vi "ZM-TST-udp.vi"() -> (0 "error out":errorcluster, 3 "Pass":bool)   [LabVIEW 2020, in "ZM-TST-tests.lvlib"]
doc: "T5, test of the UDP transport and the multi protocol: a sent package arrives unchanged, a receive with no data times out, sending with no listener is silent, a multi protocol of two file loggers writes to both, and publish on the receiver returns 5000. Pass = AND of the six checks. Side effects: UDP on 127.0.0.1:61557, two folders under output."
uses:
  ZM-TST-tests.lvlib
  protocol/ZM-CP-UDP-udp_transport/ZM-CP-UDP-receiver/ZM-CP-UDP-receiver.lvclass
  protocol/ZM-CP-UDP-udp_transport/ZM-CP-UDP-sender/ZM-CP-UDP-sender.lvclass
  protocol/ZM-CP-FL-file_logger/ZM-CP-FL-file_logger/ZM-CP-FL-file_logger.lvclass
  protocol/ZM-CP-communication_protocol/ZM-CP-communication_protocol/ZM-CP-communication_protocol.lvclass
  protocol/ZM-CP-MX-multi_protocol/ZM-CP-MX-multi_protocol/ZM-CP-MX-multi_protocol.lvclass
  common/ZM-PC-packages/ZM-PC-TP-test_package/ZM-PC-TP-test_package.lvclass
  common/ZM-PC-packages/ZM-PC-package/ZM-PC-package.lvclass
panel:
  out "rx_publish_5000_ok":bool
  out "mx_ok":bool
  out "no_listener_ok":bool
  out "timeout_ok":bool
  out "roundtrip_ok":bool
  out "rx_init_ok":bool
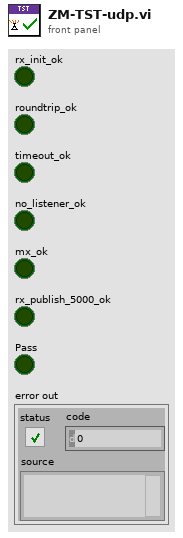
[diagram p1: front panel]
types:
  T1 = cluster{"timestamp":string, "type":string, "destination":string, "data":cluster{"temperature_c":dbl, "sample_index":i32, "duty_percent":u8, "sensor_ok":bool, "status":string}}
  T2 = enum16{"Unknown", "Root", "Hardware", "Communication"}
  T3 = cluster{"temperature_c":dbl, "sample_index":i32, "duty_percent":u8, "sensor_ok":bool, "status":string}
  T4 = cluster{"temperature_c":bool, "sample_index":bool, "duty_percent":bool, "sensor_ok":bool, "status":bool}
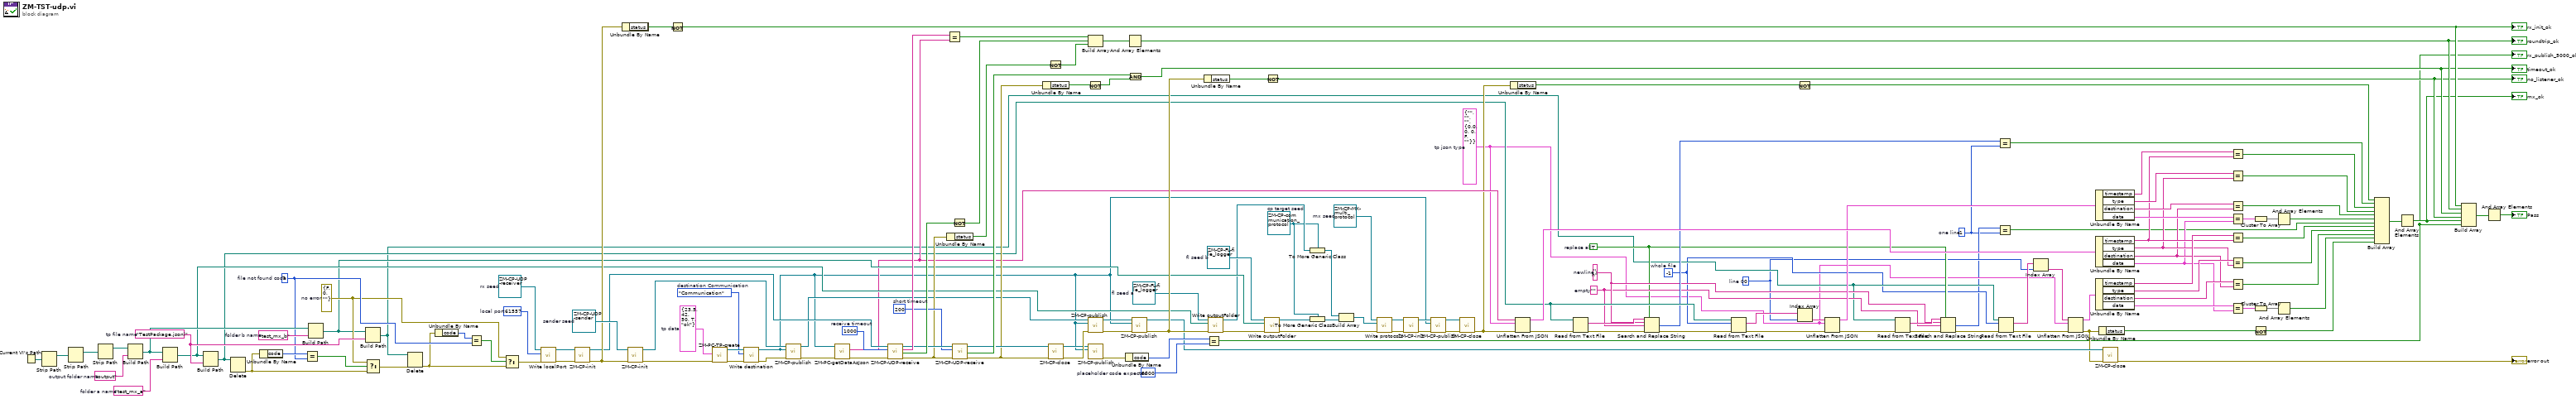
[diagram p0: block diagram]
diagram:
  w12 = 5000  # placeholder code expected
  w47 = 0  # line 0
  w41 = 1  # one line
  w50 = -1  # whole file
  w52 = TRUE  # replace all
  w54 = ""  # empty
  w55 = "\n"  # newline
  w45 = T1 {"timestamp"="", "type"="", "destination"="", "data"={"temperature_c"=0.0, "sample_index"=0, "duty_percent"=0, "sensor_ok"=FALSE, "status"=""}}  # tp json type
  w139 = errorcluster {"status"=FALSE, "code"=0, "source"=""}  # no error
  w140 = 7  # file not found code
  w146 = "TestPackage.jsonl"  # tp file name
  w147 = "test_mx_b"  # folder b name
  w149 = "test_mx_a"  # folder a name
  w150 = "output"  # output folder name
  w109 = 200  # short timeout
  w119 = 1000  # receive timeout
  w124 = T2."Communication"  # destination Communication
  w128 = T3 {"temperature_c"=23.5, "sample_index"=42, "duty_percent"=50, "sensor_ok"=TRUE, "status"="ok"}  # tp data
  w134 = u16 61557  # local port
  w86 = refnum<class "ZM-CP-MX-multi_protocol.lvclass"> refnum  # mx seed
  w89 = refnum<class "ZM-CP-communication_protocol.lvclass"> refnum  # cp target seed
  w93 = refnum<class "ZM-CP-FL-file_logger.lvclass"> refnum  # fl seed b
  w96 = refnum<class "ZM-CP-FL-file_logger.lvclass"> refnum  # fl seed a
  w130 = refnum<class "ZM-CP-UDP-sender.lvclass"> refnum  # sender seed
  w135 = refnum<class "ZM-CP-UDP-receiver.lvclass"> refnum  # rx seed
  n1 = Current VI's Path() -> (path=w154:path)
  n2 = Strip Path(path=w154) -> (stripped path=w153:path)  [unwired: 1 out]
  n3 = Strip Path(path=w153) -> (stripped path=w152:path)  [unwired: 1 out]
  n4 = Strip Path(path=w152) -> (stripped path=w151:path)  [unwired: 1 out]
  n5 = Build Path(base path=w151, name or relative path=w150) -> (appended path=w148:path)
  n6 = Build Path(base path=w148, name or relative path=w149) -> (appended path=w95:path)
  n7 = Build Path(base path=w95, name or relative path=w146) -> (appended path=w70:path)
  n8 = Delete(path (use dialog)=w70) -> (error out=w143:errorcluster)  [unwired: 4 in, 2 out]
  n9 = Unbundle By Name(w143) -> ("code"=w145:i32)
  n10 = Equal?(x=w145, y=w140) -> (x = y?=w144:bool)
  n11 = Build Path(base path=w148, name or relative path=w147) -> (appended path=w92:path)
  n12 = Build Path(base path=w92, name or relative path=w146) -> (appended path=w51:path)
  n13 = Select(t=w139, s=w144, f=w143) -> (s? t:f=w142:errorcluster)
  n14 = Delete(path (use dialog)=w51, error in=w142) -> (error out=w137:errorcluster)  [unwired: 3 in, 2 out]
  n15 = Unbundle By Name(w137) -> ("code"=w141:i32)
  n16 = Equal?(x=w141, y=w140) -> (x = y?=w138:bool)
  n17 = Select(t=w139, s=w138, f=w137) -> (s? t:f=w136:errorcluster)
  n18 = call "Write localPort.vi"("error in (no error)"=w136, "localPort"=w134, "ZM-CP-UDP-receiver in"=w135) -> ("error out"=w132:errorcluster, "ZM-CP-UDP-receiver out"=w133:refnum<class "ZM-CP-UDP-receiver.lvclass">)  [unwired: 7 in]
  n19 = call-dynamic "ZM-CP-init.vi"("error in (no error)"=w132, "ZM-CP-UDP-receiver in"=w133) -> ("error out"=w129:errorcluster, "ZM-CP-UDP-receiver out"=w120:refnum<class "ZM-CP-UDP-receiver.lvclass">)  [unwired: 8 in]
  n20 = Unbundle By Name(w129) -> ("status"=w131:bool)
  n21 = call-dynamic "ZM-CP-init.vi"("error in (no error)"=w129, "ZM-CP-UDP-sender in"=w130) -> ("error out"=w127:errorcluster, "ZM-CP-UDP-sender out"=w123:refnum<class "ZM-CP-UDP-sender.lvclass">)  [unwired: 8 in]
  n22 = Not(x=w131) -> (.not. x?=w8:bool)
  "rx_init_ok" <- w8
  n23 = call "ZM-PC-TP-create.vi"("error in (no error)"=w127, "data"=w128) -> ("error out"=w126:errorcluster, "package"=w125:refnum<class "ZM-PC-TP-test_package.lvclass">)  [unwired: 8 in]
  n24 = call "Write destination.vi"("error in (no error)"=w126, "ZM-PC-DESTINATION"=w124, "ZM-PC-package in"=w125) -> ("error out"=w122:errorcluster, "ZM-PC-package out"=w15:refnum<class "ZM-PC-TP-test_package.lvclass">)  [unwired: 7 in]
  n25 = call-dynamic "ZM-CP-publish.vi"("error in (no error)"=w122, "package"=w15, "ZM-CP-UDP-sender in"=w123) -> ("error out"=w121:errorcluster, "ZM-CP-UDP-sender out"=w102:refnum<class "ZM-CP-UDP-sender.lvclass">)  [unwired: 7 in]
  n26 = call-dynamic "ZM-PC-getDataAsJson.vi"("error in (no error)"=w121, "ZM-PC-TP-test_package in"=w15) -> ("error out"=w118:errorcluster, "json"=w76:string)  [unwired: 7 in, 1 out]
  n27 = call "ZM-CP-UDP-receive.vi"("error in (no error)"=w118, "timeout_ms"=w119, "ZM-CP-UDP-receiver in"=w120) -> ("error out"=w108:errorcluster, "timed_out"=w116:bool, "json"=w117:string, "ZM-CP-UDP-receiver out"=w110:refnum<class "ZM-CP-UDP-receiver.lvclass">)  [unwired: 5 in]
  n28 = Unbundle By Name(w108) -> ("status"=w115:bool)
  n29 = Equal?(x=w117, y=w76) -> (x = y?=w114:bool)
  n30 = Not(x=w116) -> (.not. x?=w113:bool)
  n31 = call "ZM-CP-UDP-receive.vi"("error in (no error)"=w108, "timeout_ms"=w109, "ZM-CP-UDP-receiver in"=w110) -> ("error out"=w103:errorcluster, "timed_out"=w106:bool, "ZM-CP-UDP-receiver out"=w104:refnum<class "ZM-CP-UDP-receiver.lvclass">)  [unwired: 5 in, 1 out]
  n32 = Unbundle By Name(w103) -> ("status"=w107:bool)
  n33 = Not(x=w115) -> (.not. x?=w112:bool)
  n34 = call-dynamic "ZM-CP-close.vi"("error in (no error)"=w103, "ZM-CP-UDP-receiver in"=w104) -> ("error out"=w101:errorcluster, "ZM-CP-UDP-receiver out"=w16:refnum<class "ZM-CP-UDP-receiver.lvclass">)  [unwired: 8 in]
  n35 = Not(x=w107) -> (.not. x?=w105:bool)
  n36 = Build Array(w114, w113, w112) -> (w111:bool[])
  n37 = call-dynamic "ZM-CP-publish.vi"("error in (no error)"=w101, "package"=w15, "ZM-CP-UDP-sender in"=w102) -> ("error out"=w99:errorcluster, "ZM-CP-UDP-sender out"=w100:refnum<class "ZM-CP-UDP-sender.lvclass">)  [unwired: 7 in]
  n38 = call-dynamic "ZM-CP-publish.vi"("package"=w15, "ZM-CP-communication_protocol in"=w16) -> ("error out"=w14:errorcluster)  [unwired: 8 in, 1 out]
  n39 = Unbundle By Name(w14) -> ("code"=w13:i32)
  n40 = And Array Elements(Boolean array=w111) -> (logical AND=w7:bool)
  "roundtrip_ok" <- w7
  n41 = And(x=w106, y=w105) -> (x .and. y?=w6:bool)
  "timeout_ok" <- w6
  n42 = call-dynamic "ZM-CP-publish.vi"("error in (no error)"=w99, "package"=w15, "ZM-CP-UDP-sender in"=w100) -> ("error out"=w97:errorcluster, "ZM-CP-UDP-sender out"=w11:refnum<class "ZM-CP-UDP-sender.lvclass">)  [unwired: 7 in]
  n43 = Unbundle By Name(w97) -> ("status"=w98:bool)
  n44 = Equal?(x=w13, y=w12) -> (x = y?=w3:bool)
  "rx_publish_5000_ok" <- w3
  n45 = call "Write outputFolder.vi"("error in (no error)"=w97, "outputFolder"=w95, "ZM-CP-FL-file_logger in"=w96) -> ("error out"=w94:errorcluster, "ZM-CP-FL-file_logger out"=w91:refnum<class "ZM-CP-FL-file_logger.lvclass">)  [unwired: 7 in]
  n46 = call "Write outputFolder.vi"("error in (no error)"=w94, "outputFolder"=w92, "ZM-CP-FL-file_logger in"=w93) -> ("error out"=w84:errorcluster, "ZM-CP-FL-file_logger out"=w90:refnum<class "ZM-CP-FL-file_logger.lvclass">)  [unwired: 7 in]
  n47 = Not(x=w98) -> (.not. x?=w5:bool)
  "no_listener_ok" <- w5
  n48 = To More Generic Class(target class=w89, reference=w91) -> (generic class reference=w88:refnum<class "ZM-CP-communication_protocol.lvclass">)
  n49 = To More Generic Class(target class=w89, reference=w90) -> (generic class reference=w87:refnum<class "ZM-CP-communication_protocol.lvclass">)
  n50 = Build Array(w88, w87) -> (w85:refnum<class "ZM-CP-communication_protocol.lvclass">[])
  n51 = call "Write protocols.vi"("error in (no error)"=w84, "ZM-CP-MX-PROTOCOLS"=w85, "ZM-CP-MX-multi_protocol in"=w86) -> ("error out"=w82:errorcluster, "ZM-CP-MX-multi_protocol out"=w83:refnum<class "ZM-CP-MX-multi_protocol.lvclass">)  [unwired: 7 in]
  n52 = call-dynamic "ZM-CP-init.vi"("error in (no error)"=w82, "ZM-CP-MX-multi_protocol in"=w83) -> ("error out"=w80:errorcluster, "ZM-CP-MX-multi_protocol out"=w81:refnum<class "ZM-CP-MX-multi_protocol.lvclass">)  [unwired: 8 in]
  n53 = call-dynamic "ZM-CP-publish.vi"("error in (no error)"=w80, "package"=w15, "ZM-CP-MX-multi_protocol in"=w81) -> ("error out"=w78:errorcluster, "ZM-CP-MX-multi_protocol out"=w79:refnum<class "ZM-CP-MX-multi_protocol.lvclass">)  [unwired: 7 in]
  n54 = call-dynamic "ZM-CP-close.vi"("error in (no error)"=w78, "ZM-CP-MX-multi_protocol in"=w79) -> ("error out"=w75:errorcluster)  [unwired: 8 in, 1 out]
  n55 = Unbundle By Name(w75) -> ("status"=w77:bool)
  n56 = Unflatten From JSON(JSON string=w76, type and defaults=w45, error in (no error)=w75) -> (value=w74:T1, error out=w73:errorcluster)  [unwired: 4 in]
  n57 = Read from Text File(file (use dialog)=w70, error in=w73) -> (text=w72:string, error out=w71:errorcluster)  [unwired: 2 in, 2 out]
  n58 = Search and Replace String(replace all?=w52, input string=w72, search string=w55, replace string=w54, error in=w71) -> (number of replacements=w64:i32, error out=w69:errorcluster)  [unwired: 3 in, 2 out]
  n59 = Read from Text File(file (use dialog)=w70, count=w50, error in=w69) -> (text=w68:string[], error out=w66:errorcluster)  [unwired: 1 in, 2 out]
  n60 = Not(x=w77) -> (.not. x?=w29:bool)
  n61 = Index Array(array=w68, index=w47) -> (element=w67:string)
  n62 = Unflatten From JSON(JSON string=w67, type and defaults=w45, error in (no error)=w66) -> (value=w65:T1, error out=w57:errorcluster)  [unwired: 4 in]
  n63 = Read from Text File(file (use dialog)=w51, error in=w57) -> (text=w56:string, error out=w53:errorcluster)  [unwired: 2 in, 2 out]
  n64 = Search and Replace String(replace all?=w52, input string=w56, search string=w55, replace string=w54, error in=w53) -> (number of replacements=w42:i32, error out=w49:errorcluster)  [unwired: 3 in, 2 out]
  n65 = Equal?(x=w64, y=w41) -> (x = y?=w28:bool)
  n66 = Equal?(x=w42, y=w41) -> (x = y?=w23:bool)
  n67 = Read from Text File(file (use dialog)=w51, count=w50, error in=w49) -> (text=w48:string[], error out=w44:errorcluster)  [unwired: 1 in, 2 out]
  n68 = Index Array(array=w48, index=w47) -> (element=w46:string)
  n69 = Unflatten From JSON(JSON string=w46, type and defaults=w45, error in (no error)=w44) -> (value=w43:T1, error out=w10:errorcluster)  [unwired: 4 in]
  n70 = Unbundle By Name(w65) -> ("timestamp"=w63:string, "type"=w62:string, "destination"=w61:string, "data"=w60:T3)
  n71 = Unbundle By Name(w74) -> ("timestamp"=w39:string, "type"=w37:string, "destination"=w35:string, "data"=w33:T3)
  n72 = Unbundle By Name(w43) -> ("timestamp"=w40:string, "type"=w38:string, "destination"=w36:string, "data"=w34:T3)
  n73 = Unbundle By Name(w10) -> ("status"=w30:bool)
  n74 = call-dynamic "ZM-CP-close.vi"("error in (no error)"=w10, "ZM-CP-UDP-sender in"=w11) -> ("error out"=→"error out":errorcluster)  [unwired: 8 in, 1 out]
  n75 = Equal?(x=w63, y=w39) -> (x = y?=w27:bool)
  n76 = Equal?(x=w62, y=w37) -> (x = y?=w26:bool)
  n77 = Equal?(x=w61, y=w35) -> (x = y?=w25:bool)
  n78 = Equal?(x=w60, y=w33) -> (x = y?=w59:T4)
  n79 = Equal?(x=w40, y=w39) -> (x = y?=w22:bool)
  n80 = Equal?(x=w38, y=w37) -> (x = y?=w21:bool)
  n81 = Equal?(x=w36, y=w35) -> (x = y?=w20:bool)
  n82 = Equal?(x=w34, y=w33) -> (x = y?=w32:T4)
  n83 = Cluster To Array(cluster=w59) -> (array=w58:bool[])
  n84 = Cluster To Array(cluster=w32) -> (array=w31:bool[])
  n85 = Not(x=w30) -> (.not. x?=w18:bool)
  n86 = And Array Elements(Boolean array=w58) -> (logical AND=w24:bool)
  n87 = And Array Elements(Boolean array=w31) -> (logical AND=w19:bool)
  n88 = Build Array(w29, w28, w27, w26, w25, w24, w23, w22, w21, w20, w19, w18) -> (w17:bool[])
  n89 = And Array Elements(Boolean array=w17) -> (logical AND=w4:bool)
  "mx_ok" <- w4
  n90 = Build Array(w8, w7, w6, w5, w4, w3) -> (w9:bool[])
  n91 = And Array Elements(Boolean array=w9) -> (logical AND=→"Pass":bool)
